vi "Parse Amount.vi"(8 "error in":errorcluster, 11 "User Input":string) -> (0 "error out":errorcluster, 2 "Amount":dbl, 3 "Valid Amount?":bool)   [LabVIEW 2026]
doc: "Converts the text the user typed into a money amount. Leading and trailing whitespace is removed, then the whole remaining text must be one number with a period as decimal separator (independent of the system locale), finite and greater than zero. Valid Amount? is TRUE and Amount carries the number when it is; otherwise Valid Amount? is FALSE and Amount is 0. Invalid input is NOT an error - error in is passed through to error out unchanged so the caller can show a message. No file access."
uses:
  <vilib>/Utility/error.llb/Trim Whitespace (string).vi
  <vilib>/Utility/error.llb/Trim Whitespace One-Sided.vi
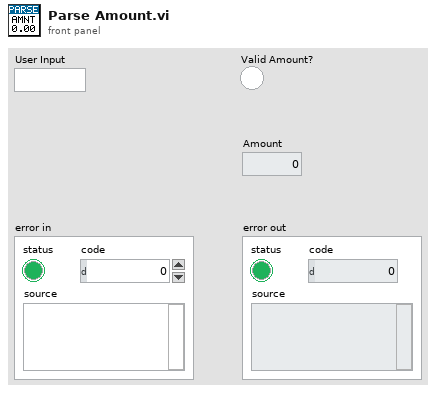
[diagram p1: front panel]
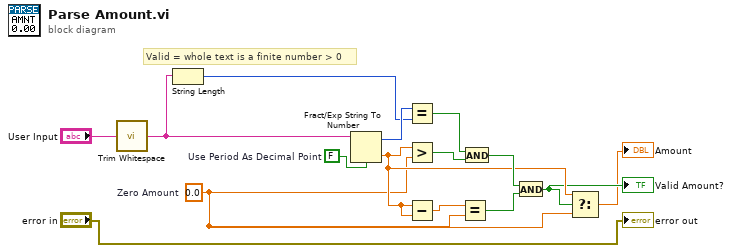
[diagram p0: block diagram]
diagram:
  w4 = 0.0  # Zero Amount
  w14 = FALSE  # Use Period As Decimal Point
  # "Valid = whole text is a finite number > 0"
  n1 = call-poly <vilib>:"Trim Whitespace.vi"("string"="User Input") -> ("trimmed string"=w13:string)  [unwired: 1 in]
  n2 = String Length(string=w13) -> (length=w11:i32)
  n3 = Fract/Exp String To Number(use system decimal point (T)=w14, string=w13) -> (offset past number=w12:i32, number=w5:dbl)  [unwired: 2 in]
  n4 = Equal?(x=w12, y=w11) -> (x = y?=w9:bool)
  n5 = Greater?(x=w5, y=w4) -> (0:w8:bool)
  n6 = Subtract(x=w5, y=w5) -> (x-y=w10:dbl)
  n7 = Equal?(x=w10, y=w4) -> (x = y?=w6:bool)
  n8 = And(x=w9, y=w8) -> (x .and. y?=w7:bool)
  n9 = And(x=w7, y=w6) -> (x .and. y?=w3:bool)
  "Valid Amount?" <- w3
  n10 = Select(t=w5, s=w3, f=w4) -> (s? t:f=→"Amount":dbl)
  "error out" <- "error in"
